vi "NLTest.vi"() -> ()   [LabVIEW 2017, in "NLTest.lvclass"]
uses:
  NLTestCLASS/NLTest.lvclass
  NLTestCLASS/NLT-seqeditor.ctl
panel:
  in  "序列编辑":T1
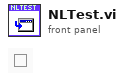
[diagram p1: front panel]
types:
  T1 = typedef "NLTest.lvclass/NLT-seqeditor.ctl" = bool
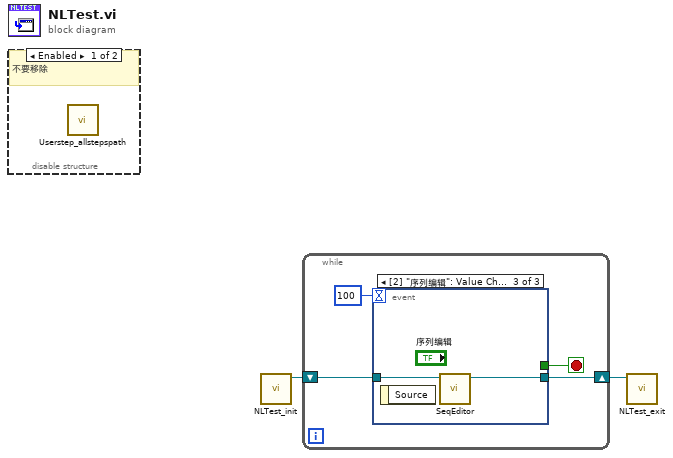
[diagram p0: block diagram]
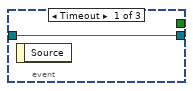
[diagram p3: hidden frame]
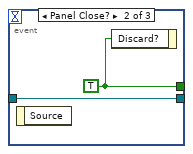
[diagram p4: hidden frame]
diagram:
  n1 = disable-structure shown="Enabled" {
    frame Enabled {
      # "不要移除"
      n2 = call "Userstep_allstepspath.vi"() -> ()  [unwired: 11 in, 1 out]
    }
    frame Disabled {
    }
  }
  n3 = call "NLTest_init.vi"() -> ("NLTest out"=w2:refnum<class "NLTest.lvclass">)  [unwired: 10 in, 1 out]
  n4 = while {
    shift-right: [w3] -> w1
    shift-left: w2 -> [w4]
    stop <- w5 stop-if-true
    n5 = event shown="[2] \"序列编辑\": Value Change" {
      selector: _ -> [_ _ _]
      dyn-events: _ -> [_ _ _]
      timeout: 100 -> [_ _ _]
      tunnel: [_ w9 _] -> w5
      tunnel: [w7 w8 w11] -> w3
      tunnel: w4 -> [w7 w8 w10]
      event Timeout {
        n6 = event-data() -> ()  [unwired: 1 in, 1 out]
      }
      event Panel Close? {
        w9 = TRUE ("Discard?")
        n7 = event-data() -> ()  [unwired: 1 in, 1 out]
        n8 = event-data("Discard?"=w9) -> ()  [unwired: 1 in, 1 out]
      }
      event Value Change {
        n9 = event-data() -> ()  [unwired: 1 in, 1 out]
        n10 = call "SeqEditor.vi"("NLTest in"=w10) -> ("NLTest out"=w11:refnum<class "NLTest.lvclass">)  [unwired: 9 in, 1 out]
      }
    }
  }
  n11 = call "NLTest_exit.vi"("NLTest in"=w1) -> ()  [unwired: 10 in, 1 out]
